vi "ReadPAQdata.vi"(4 "Tags":string[](array[string]), 6 "TableName":string, 8 "error in (no error)":errorcluster, 9 "Time-End":timestamp, 10 "Time-Start":timestamp, 11 "DBAL-BIN in":refnum<class "DBAL-BIN.lvclass">) -> (0 "error out":errorcluster, 2 "PAQ_section":T1, 3 "DBAL-BIN out":refnum<class "DBAL-BIN.lvclass">)   [LabVIEW 2020, in "Sgraph_lib_V1.lvlib" / "DBAL-BIN.lvclass"]
doc: "Andre Koelewijn, 8 May 2021,\n\nRead a PAQ TAGs from the BIN database for a defined time span.\nThe Layer input defines from which layer the data should be read."
uses:
  DBAL-BIN.lvclass
  controls/BIN/BINdata.ctl
  DBAL-BIN.lvclass/DBAL-BIN.ctl
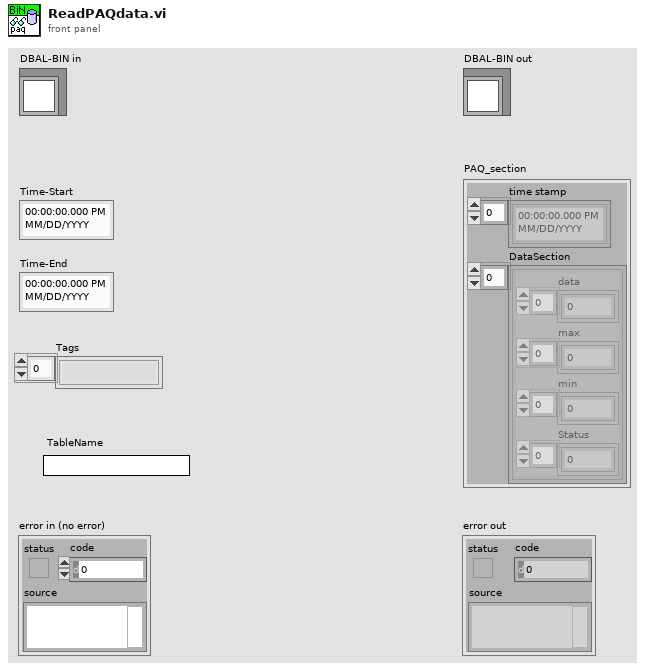
[diagram p1: front panel]
types:
  T1 = cluster{"time stamp":timestamp[], "DataSection":cluster{"data":dbl[], "max":dbl[], "min":dbl[], "Status":u32[]}[]}
  T2 = typedef "Sgraph_lib_V1.lvlib/DBAL-BIN.lvclass/BINdata.ctl" = cluster{"time":dbl[], "TagsData":cluster{"data":dbl[], "max":dbl[], "min":dbl[], "status":u32[]}[]}
  T3 = typedef "Sgraph_lib_V1.lvlib/DBAL-BIN.lvclass/BinFolderPace.ctl" = enum16{"PerDay", "PerWeek", "PerYear"}
  T4 = cluster{"Seq":i32, "Start":timestamp, "Stop":timestamp}[]
  T5 = cluster{"data":dbl[], "max":dbl[], "min":dbl[], "status":u32[]}[]
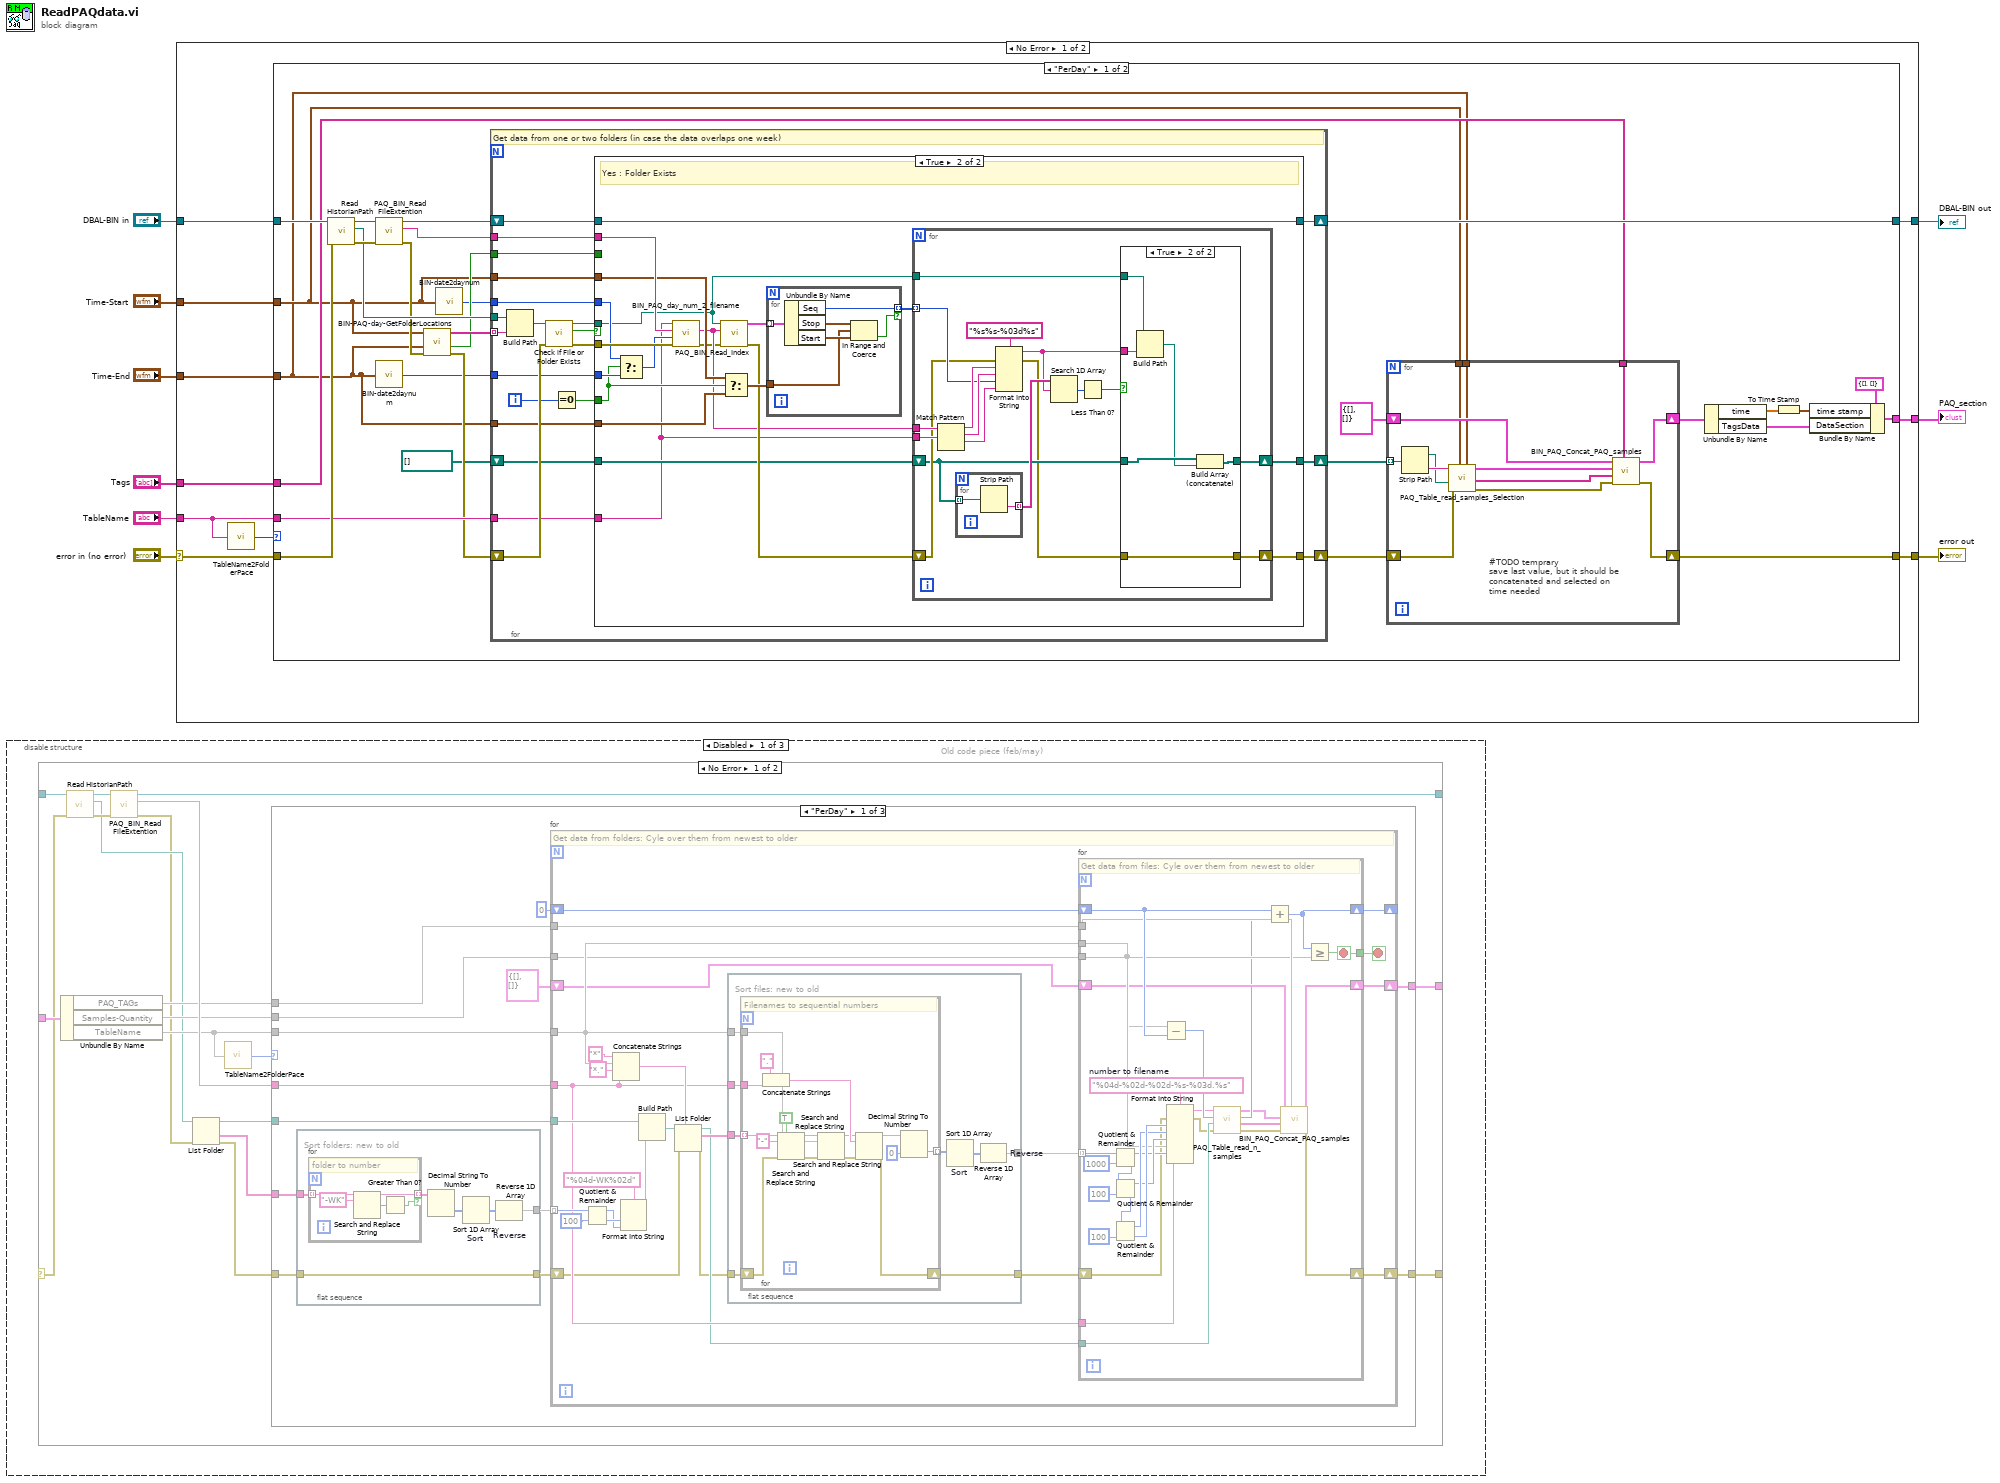
[diagram p0: block diagram]
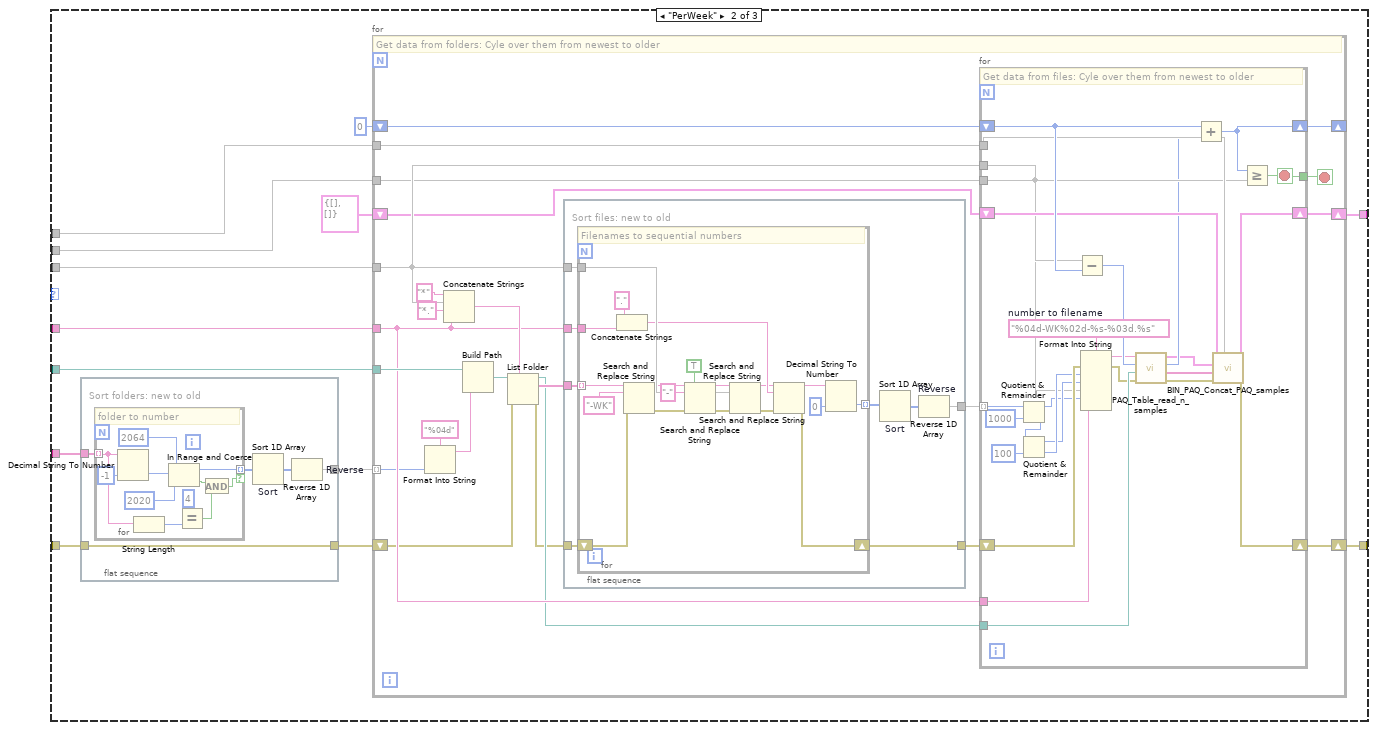
[diagram p2: hidden frame]
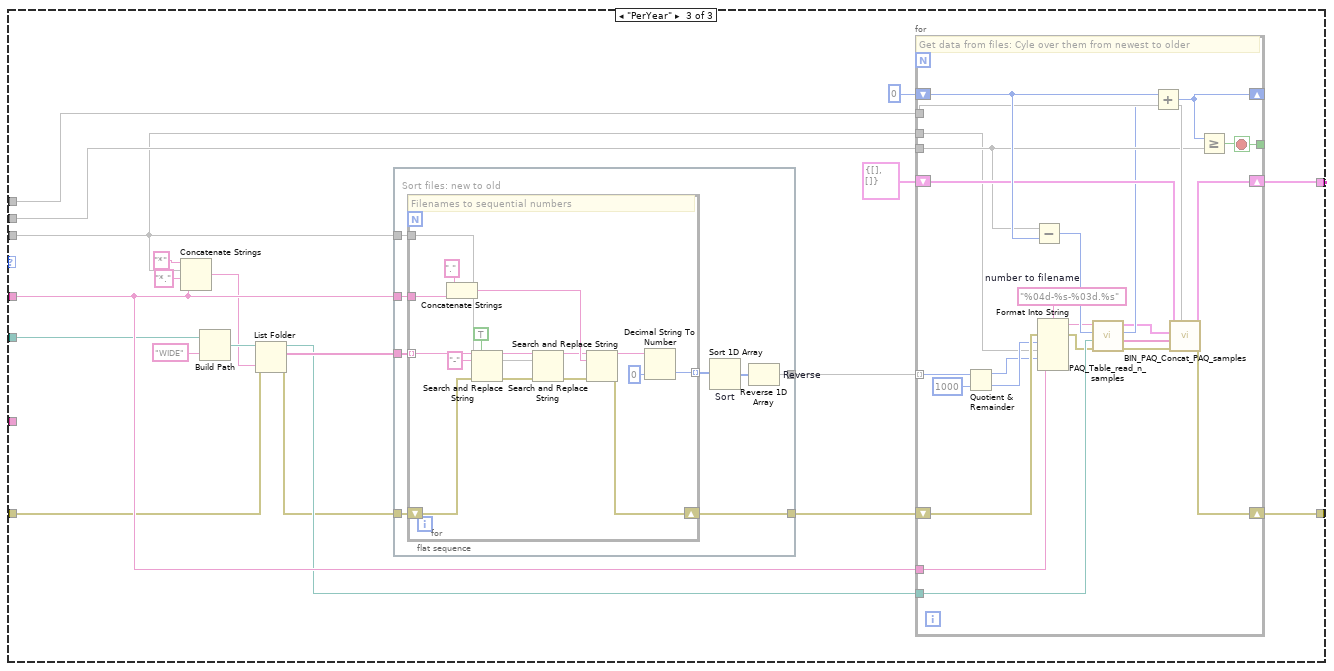
[diagram p3: hidden frame]
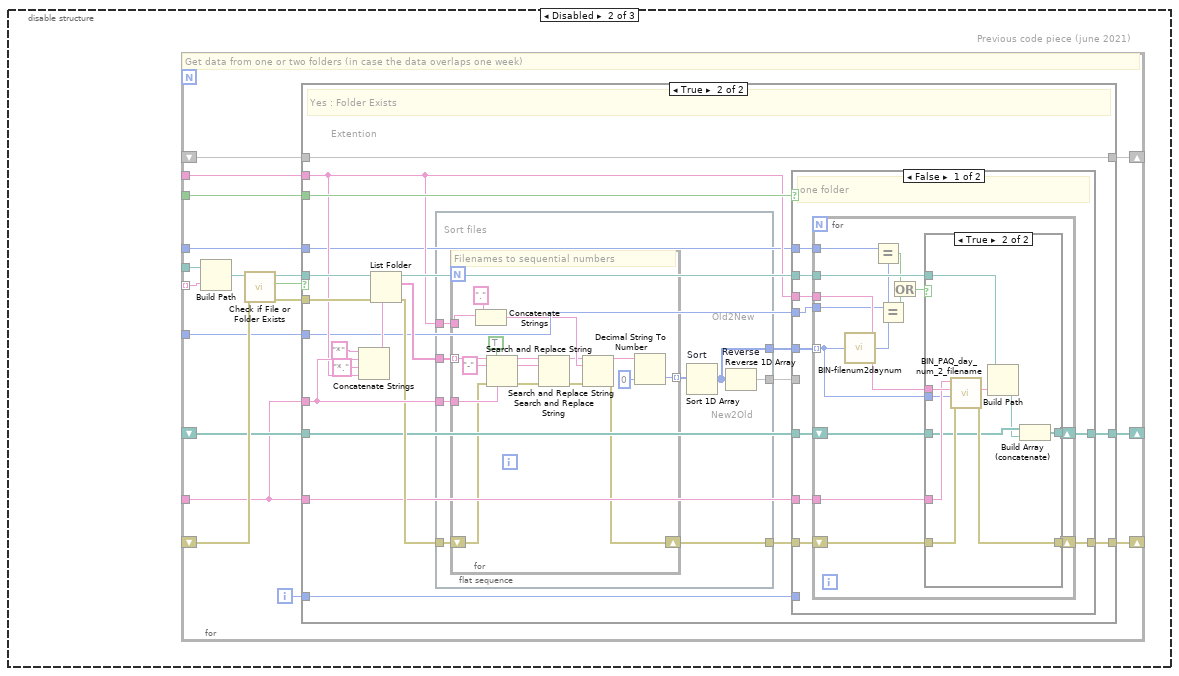
[diagram p5: hidden frame]
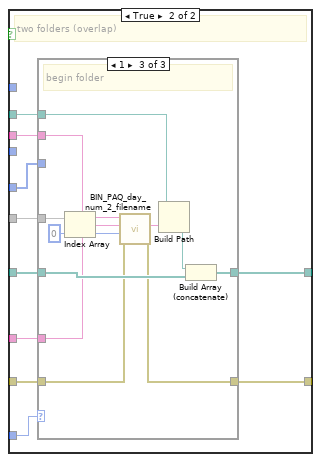
[diagram p8: hidden frame]
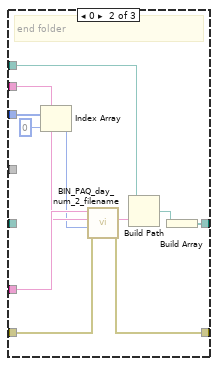
[diagram p10: hidden frame]
diagram:
  n1 = disable-structure shown="Disabled" {
    frame Disabled {
      # "Old code piece (feb/may)"
      n2 = case shown="No Error" {
        selector: _ -> [w22 w308]
        tunnel: [w26 w308] -> _
        tunnel: _ -> [w23 w309]
        tunnel: [w19 w309] -> _
        tunnel: _ -> [w27 _]
        tunnel: [w17 _] -> _
        frame No Error {
          n3 = Unbundle By Name(w27) -> ("PAQ_TAGs"=w18, "Samples-Quantity"=w20, "TableName"=w16)
          n4 = call "Read HistorianPath.vi"("error in (no error)"=w22, "DBAL-BIN in"=w23) -> ("error out"=w21:errorcluster, "HistorianPath"=w14:path, "DBAL-BIN out"=w24:refnum<class "DBAL-BIN.lvclass">)  [unwired: 7 in]
          n5 = call "PAQ_BIN_Read FileExtention.vi"("error in (no error)"=w21, "DBAL-BIN in"=w24) -> ("error out"=w13:errorcluster, "FileExtention"=w25:string, "DBAL-BIN out"=w19:refnum<class "DBAL-BIN.lvclass">)  [unwired: 7 in]
          n6 = List Folder(path=w14, error in=w13) -> (path out=w10:path, folder names=w12:string[], error out=w11:errorcluster)  [unwired: 2 in, 1 out]
          n7 = call "TableName2FolderPace.vi"("TableName"=w16) -> ("FolderPace"=w15:T3)  [unwired: 6 in]
          n8 = case shown="\"PerDay\"" w15 {
            tunnel: [w40 w145 w259] -> w26
            tunnel: w25 -> [w39 w144 w258]
            tunnel: w20 -> [w38 w143 w257]
            tunnel: w18 -> [w36 w141 w256]
            tunnel: [w34 w139 w254] -> w17
            tunnel: w16 -> [w33 w138 w253]
            tunnel: w12 -> [w32 w137 _]
            tunnel: w11 -> [w30 w135 w240]
            tunnel: w10 -> [w29 w134 w252]
            frame "PerDay" {
              n9 = flat-sequence {
                tunnel: w32 -> [w46]
                tunnel: [w41] -> w28
                tunnel: w30 -> [w43]
                tunnel: [w43] -> w31
                frame #0 {
                  # "Sort folders: new to old"
                  n10 = for {
                    tunnel: w46 -> [w51] mode=indexing
                    tunnel: [w49] -> w45 mode=indexing if=w47
                    # "folder to number"
                    n11 = Search and Replace String(input string=w51, search string="-WK") -> (result string=w49:string, number of replacements=w48:i32)  [unwired: 6 in, 2 out]
                    n12 = Greater Than 0?(x=w48) -> (x > 0?=w47:bool)
                  }
                  n13 = Decimal String To Number ("to num")(string=w45) -> (number=w44:i32[])  [unwired: 2 in, 1 out]
                  n14 = Sort 1D Array "Sort"(array=w44) -> (sorted array=w42:i32[])
                  n15 = Reverse 1D Array "Reverse"(array=w42) -> (reversed array=w41:i32[])
                }
              }
              n16 = for {
                shift-right: [w62] -> w40
                shift-left: w31 -> [w53]
                tunnel: w28 -> [w78] mode=indexing
                tunnel: w39 -> [w65]
                tunnel: w29 -> [w73]
                tunnel: w33 -> [w66]
                tunnel: w38 -> [w61]
                shift-right: [w59] -> _
                shift-left: 0 ("Fetched samples") -> [w60]
                tunnel: w36 -> [w58]
                shift-right: [w57] -> w34
                shift-left: T2 {"time"=[], "TagsData"=[]} ("BinHistData") -> [w56]
                stop <- w55 stop-if-true
                # "Get data from folders: Cyle over them from newest to older"
                n17 = Quotient & Remainder(x=w78, y=100) -> (x-y*floor(x/y)=w74:i32, floor(x/y)=w75:i32)
                n18 = Concatenate Strings("*", w66, "*.", w65) -> (w69:string)
                n19 = Format Into String(format string="%04d-WK%02d", w75, w74) -> (resulting string=w54:string)  [unwired: 2 in, 1 out]
                n20 = Build Path(base path=w73, name or relative path=w54) -> (appended path=w72:path)
                n21 = List Folder(path=w72, pattern=w69, error in=w53) -> (path out=w64:path, filenames=w67:string[], error out=w52:errorcluster)  [unwired: 1 in, 1 out]
                n22 = flat-sequence {
                  tunnel: w67 -> [w116]
                  tunnel: w66 -> [w115]
                  tunnel: w65 -> [w114]
                  tunnel: [w111] -> w68
                  tunnel: w52 -> [w110]
                  tunnel: [w109] -> w63
                  frame #0 {
                    # "Sort files: new to old"
                    n23 = for {
                      tunnel: w116 -> [w121] mode=indexing
                      tunnel: w115 -> [w129]
                      tunnel: w114 -> [w128]
                      tunnel: [w123] -> w112 mode=indexing
                      shift-right: [w117] -> w109
                      shift-left: w110 -> [w120]
                      # "Filenames to sequential numbers"
                      n24 = Concatenate Strings("." ("string"), w128) -> (w127:string)
                      n25 = Search and Replace String(replace all?=TRUE ("replace all? (F)"), input string=w121, search string="-", error in=w120) -> (result string=w130:string, error out=w119:errorcluster)  [unwired: 4 in, 2 out]
                      n26 = Search and Replace String(input string=w130, search string=w129, error in=w119) -> (result string=w126:string, error out=w118:errorcluster)  [unwired: 5 in, 2 out]
                      n27 = Search and Replace String(input string=w126, search string=w127, error in=w118) -> (result string=w124:string, error out=w117:errorcluster)  [unwired: 5 in, 2 out]
                      n28 = Decimal String To Number(string=w124, default (0L)=u64 0 ("default (0 I32)")) -> (number=w123:u64)  [unwired: 1 in, 1 out]
                    }
                    n29 = Sort 1D Array "Sort"(array=w112) -> (sorted array=w113:u64[])
                    n30 = Reverse 1D Array "Reverse"(array=w113) -> (reversed array=w111:u64[])
                  }
                }
                n31 = for {
                  tunnel: w68 -> [w107] mode=indexing
                  tunnel: w66 -> [w98]
                  tunnel: w65 -> [w96]
                  tunnel: w64 -> [w94]
                  shift-right: [w87] -> w62
                  shift-left: w63 -> [w95]
                  tunnel: w61 -> [w84]
                  shift-right: [w80] -> w59
                  shift-left: w60 -> [w91]
                  tunnel: w58 -> [w85]
                  shift-right: [w89] -> w57
                  shift-left: w56 -> [w90]
                  tunnel: [w83] -> w55
                  stop <- w83 stop-if-true
                  w102 = "%04d-%02d-%02d-%s-%03d.%s"  # number to filename
                  # "Get data from files: Cyle over them from newest to older"
                  n32 = Quotient & Remainder(x=w107, y=u64 1000) -> (x-y*floor(x/y)=w97:u64, floor(x/y)=w105:u64)
                  n33 = Quotient & Remainder(x=w105, y=u64 100) -> (x-y*floor(x/y)=w99:u64, floor(x/y)=w103:u64)
                  n34 = Quotient & Remainder(x=w103, y=u64 100) -> (x-y*floor(x/y)=w100:u64, floor(x/y)=w101:u64)
                  n35 = Subtract(x=w84, y=w91) -> (x-y=w92:i32)
                  n36 = Format Into String(format string=w102, error in=w95, w101, w100, w99, w98, w97, w96) -> (resulting string=w79:string, error out=w93:errorcluster)  [unwired: 1 in]
                  n37 = call "PAQ_Table_read_n_samples.vi"("error in (no error)"=w93, "Sub Path"=w94, "Required samples"=w92, "Table Filename"=w79) -> ("error out"=w88:errorcluster, "TAGs"=w86:string[], "Fetched samples"=w82:i32, "value"=w81:T2)  [unwired: 4 in]
                  n38 = Add(x=w91, y=w82) -> (x+y=w80:i32)
                  n39 = call "BIN_PAQ_Concat_PAQ_samples.vi"("Memory TAGs"=w85, "error in (no error)"=w88, "Added samples TAGs"=w86, "PAQ Samples to ADD"=w81, "PAQ Samples IN"=w90) -> ("error out"=w87:errorcluster, "PAQ Samples OUT"=w89:T2)  [unwired: 5 in]
                  n40 = Greater Or Equal?(x=w80, y=w84) -> (x >= y?=w83:bool)
                }
              }
            }
            frame "PerWeek" {
              n41 = flat-sequence {
                tunnel: w137 -> [w150]
                tunnel: [w147] -> w133
                tunnel: w135 -> [w149]
                tunnel: [w149] -> w136
                frame #0 {
                  # "Sort folders: new to old"
                  n42 = for {
                    tunnel: w150 -> [w156] mode=indexing
                    tunnel: [w157] -> w146 mode=indexing if=w151
                    # "folder to number"
                    n43 = Decimal String To Number ("to num")(string=w156, default (0L)=-1 ("default (0 I32)")) -> (number=w160:i32)  [unwired: 1 in, 1 out]
                    n44 = String Length(string=w156) -> (length=w155:i32)
                    n45 = In Range and Coerce(upper limit=2064 ("lower limit"), x=w160, lower limit=2020) -> (coerced(x)=w157:i32, In Range?=w153:bool)
                    n46 = Equal?(x=4, y=w155) -> (x = y?=w152:bool)
                    n47 = And(x=w153, y=w152) -> (x .and. y?=w151:bool)
                  }
                  n48 = Sort 1D Array "Sort"(array=w146) -> (sorted array=w148:i32[])
                  n49 = Reverse 1D Array "Reverse"(array=w148) -> (reversed array=w147:i32[])
                }
              }
              n50 = for {
                shift-right: [w173] -> w145
                shift-left: w136 -> [w163]
                tunnel: w133 -> [w164] mode=indexing
                tunnel: w144 -> [w176]
                tunnel: w134 -> [w184]
                tunnel: w138 -> [w177]
                tunnel: w143 -> [w172]
                shift-right: [w170] -> _
                shift-left: 0 ("Fetched samples") -> [w171]
                tunnel: w141 -> [w169]
                shift-right: [w168] -> w139
                shift-left: T2 {"time"=[], "TagsData"=[]} ("BinHistData") -> [w167]
                stop <- w166 stop-if-true
                # "Get data from folders: Cyle over them from newest to older"
                n51 = Format Into String(format string="%04d", w164) -> (resulting string=w165:string)  [unwired: 2 in, 1 out]
                n52 = Concatenate Strings("*", w177, "*.", w176) -> (w180:string)
                n53 = Build Path(base path=w184, name or relative path=w165) -> (appended path=w183:path)
                n54 = List Folder(path=w183, pattern=w180, error in=w163) -> (path out=w175:path, filenames=w178:string[], error out=w162:errorcluster)  [unwired: 1 in, 1 out]
                n55 = flat-sequence {
                  tunnel: w178 -> [w220]
                  tunnel: w177 -> [w219]
                  tunnel: w176 -> [w218]
                  tunnel: [w215] -> w179
                  tunnel: w162 -> [w214]
                  tunnel: [w213] -> w174
                  frame #0 {
                    # "Sort files: new to old"
                    n56 = for {
                      tunnel: w220 -> [w229] mode=indexing
                      tunnel: w219 -> [w237]
                      tunnel: w218 -> [w236]
                      tunnel: [w231] -> w216 mode=indexing
                      shift-right: [w221] -> w213
                      shift-left: w214 -> [w225]
                      # "Filenames to sequential numbers"
                      n57 = Concatenate Strings("." ("string"), w236) -> (w235:string)
                      n58 = Search and Replace String(input string=w229, search string="-WK", error in=w225) -> (result string=w227:string, error out=w224:errorcluster)  [unwired: 5 in, 2 out]
                      n59 = Search and Replace String(replace all?=TRUE ("replace all? (F)"), input string=w227, search string="-", error in=w224) -> (result string=w238:string, error out=w223:errorcluster)  [unwired: 4 in, 2 out]
                      n60 = Search and Replace String(input string=w238, search string=w237, error in=w223) -> (result string=w234:string, error out=w222:errorcluster)  [unwired: 5 in, 2 out]
                      n61 = Search and Replace String(input string=w234, search string=w235, error in=w222) -> (result string=w232:string, error out=w221:errorcluster)  [unwired: 5 in, 2 out]
                      n62 = Decimal String To Number(string=w232, default (0L)=u64 0 ("default (0 I32)")) -> (number=w231:u64)  [unwired: 1 in, 1 out]
                    }
                    n63 = Sort 1D Array "Sort"(array=w216) -> (sorted array=w217:u64[])
                    n64 = Reverse 1D Array "Reverse"(array=w217) -> (reversed array=w215:u64[])
                  }
                }
                n65 = for {
                  tunnel: w179 -> [w211] mode=indexing
                  tunnel: w177 -> [w189]
                  tunnel: w176 -> [w187]
                  tunnel: w175 -> [w206]
                  shift-right: [w199] -> w173
                  shift-left: w174 -> [w207]
                  tunnel: w172 -> [w196]
                  shift-right: [w192] -> w170
                  shift-left: w171 -> [w203]
                  tunnel: w169 -> [w197]
                  shift-right: [w201] -> w168
                  shift-left: w167 -> [w202]
                  tunnel: [w195] -> w166
                  stop <- w195 stop-if-true
                  w208 = "%04d-WK%02d-%s-%03d.%s"  # number to filename
                  # "Get data from files: Cyle over them from newest to older"
                  n66 = Quotient & Remainder(x=w211, y=u64 1000) -> (x-y*floor(x/y)=w188:u64, floor(x/y)=w209:u64)
                  n67 = Quotient & Remainder(x=w209, y=u64 100) -> (x-y*floor(x/y)=w190:u64, floor(x/y)=w191:u64)
                  n68 = Subtract(x=w196, y=w203) -> (x-y=w204:i32)
                  n69 = Format Into String(format string=w208, error in=w207, w191, w190, w189, w188, w187) -> (resulting string=w186:string, error out=w205:errorcluster)  [unwired: 1 in]
                  n70 = call "PAQ_Table_read_n_samples.vi"("error in (no error)"=w205, "Sub Path"=w206, "Required samples"=w204, "Table Filename"=w186) -> ("error out"=w200:errorcluster, "TAGs"=w198:string[], "Fetched samples"=w194:i32, "value"=w193:T2)  [unwired: 4 in]
                  n71 = Add(x=w203, y=w194) -> (x+y=w192:i32)
                  n72 = call "BIN_PAQ_Concat_PAQ_samples.vi"("Memory TAGs"=w197, "error in (no error)"=w200, "Added samples TAGs"=w198, "PAQ Samples to ADD"=w193, "PAQ Samples IN"=w202) -> ("error out"=w199:errorcluster, "PAQ Samples OUT"=w201:T2)  [unwired: 5 in]
                  n73 = Greater Or Equal?(x=w192, y=w196) -> (x >= y?=w195:bool)
                }
              }
            }
            frame "PerYear" {
              n74 = Concatenate Strings("*", w253, "*.", w258) -> (w248:string)
              n75 = Build Path(base path=w252, name or relative path="WIDE" ("format string")) -> (appended path=w251:path)
              n76 = List Folder(path=w251, pattern=w248, error in=w240) -> (path out=w245:path, filenames=w246:string[], error out=w241:errorcluster)  [unwired: 1 in, 1 out]
              n77 = flat-sequence {
                tunnel: w246 -> [w291]
                tunnel: w253 -> [w290]
                tunnel: w258 -> [w289]
                tunnel: [w286] -> w247
                tunnel: w241 -> [w285]
                tunnel: [w284] -> w244
                frame #0 {
                  # "Sort files: new to old"
                  n78 = for {
                    tunnel: w291 -> [w292] mode=indexing
                    tunnel: w290 -> [w305]
                    tunnel: w289 -> [w304]
                    tunnel: [w299] -> w287 mode=indexing
                    shift-right: [w294] -> w284
                    shift-left: w285 -> [w293]
                    # "Filenames to sequential numbers"
                    n79 = Concatenate Strings("." ("string"), w304) -> (w303:string)
                    n80 = Search and Replace String(replace all?=TRUE ("replace all? (F)"), input string=w292, search string="-", error in=w293) -> (result string=w306:string, error out=w296:errorcluster)  [unwired: 4 in, 2 out]
                    n81 = Search and Replace String(input string=w306, search string=w305, error in=w296) -> (result string=w302:string, error out=w295:errorcluster)  [unwired: 5 in, 2 out]
                    n82 = Search and Replace String(input string=w302, search string=w303, error in=w295) -> (result string=w300:string, error out=w294:errorcluster)  [unwired: 5 in, 2 out]
                    n83 = Decimal String To Number(string=w300, default (0L)=u64 0 ("default (0 I32)")) -> (number=w299:u64)  [unwired: 1 in, 1 out]
                  }
                  n84 = Sort 1D Array "Sort"(array=w287) -> (sorted array=w288:u64[])
                  n85 = Reverse 1D Array "Reverse"(array=w288) -> (reversed array=w286:u64[])
                }
              }
              n86 = for {
                tunnel: w247 -> [w282] mode=indexing
                tunnel: w253 -> [w262]
                tunnel: w258 -> [w260]
                tunnel: w245 -> [w279]
                shift-right: [w272] -> w259
                shift-left: w244 -> [w280]
                tunnel: w257 -> [w269]
                shift-right: [w265] -> _
                shift-left: 0 ("Fetched samples") -> [w276]
                tunnel: w256 -> [w270]
                shift-right: [w274] -> w254
                shift-left: T2 {"time"=[], "TagsData"=[]} ("BinHistData") -> [w275]
                tunnel: [w268] -> _
                stop <- w268 stop-if-true
                w281 = "%04d-%s-%03d.%s"  # number to filename
                # "Get data from files: Cyle over them from newest to older"
                n87 = Quotient & Remainder(x=w282, y=u64 1000) -> (x-y*floor(x/y)=w261:u64, floor(x/y)=w263:u64)
                n88 = Subtract(x=w269, y=w276) -> (x-y=w277:i32)
                n89 = Format Into String(format string=w281, error in=w280, w263, w262, w261, w260) -> (resulting string=w264:string, error out=w278:errorcluster)  [unwired: 1 in]
                n90 = call "PAQ_Table_read_n_samples.vi"("error in (no error)"=w278, "Sub Path"=w279, "Required samples"=w277, "Table Filename"=w264) -> ("error out"=w273:errorcluster, "TAGs"=w271:string[], "Fetched samples"=w267:i32, "value"=w266:T2)  [unwired: 4 in]
                n91 = Add(x=w276, y=w267) -> (x+y=w265:i32)
                n92 = call "BIN_PAQ_Concat_PAQ_samples.vi"("Memory TAGs"=w270, "error in (no error)"=w273, "Added samples TAGs"=w271, "PAQ Samples to ADD"=w266, "PAQ Samples IN"=w275) -> ("error out"=w272:errorcluster, "PAQ Samples OUT"=w274:T2)  [unwired: 5 in]
                n93 = Greater Or Equal?(x=w265, y=w269) -> (x >= y?=w268:bool)
              }
            }
          }
        }
        frame Error {
        }
      }
    }
    frame Disabled {
      # "Previous code piece (june 2021)"
      n94 = for {
        shift-right: [w320] -> _
        shift-left: _ -> [w324]
        shift-right: [w321] -> _
        shift-left: _ -> [w322]
        tunnel: _ -> [w326] mode=indexing
        tunnel: _ -> [w312]
        tunnel: _ -> [w327]
        tunnel: _ -> [w319]
        tunnel: _ -> [w316]
        shift-right: [w314] -> _
        shift-left: _ -> [w313]
        tunnel: _ -> [w310]
        tunnel: _ -> [w311]
        i -> [w315]
        # "Get data from one or two folders (in case the data overlaps one week)"
        n95 = Build Path(base path=w327, name or relative path=w326) -> (appended path=w325:path)
        n96 = call <vilib>:"Check if File or Folder Exists.vi"("error in (no error)"=w324, "path"=w325) -> ("error out"=w317:errorcluster, "file or folder exists?"=w323:bool, "dup path"=w318:path)  [unwired: 7 in]
        n97 = case shown="True" w323 {
          tunnel: w322 -> [w330 w352]
          tunnel: [w330 w352] -> w321
          tunnel: [w329 w336] -> w320
          tunnel: w312 -> [_ w345]
          tunnel: w319 -> [_ w334]
          tunnel: w318 -> [_ w348]
          tunnel: w317 -> [w329 w347]
          tunnel: w316 -> [_ w343]
          tunnel: w315 -> [_ w342]
          tunnel: [w328 w333] -> w314
          tunnel: w313 -> [w328 w339]
          tunnel: w312 -> [_ w335]
          tunnel: w311 -> [_ w332]
          tunnel: w310 -> [_ w331]
          frame False {
            # "No: Folder not found"
          }
          frame True {
            # "Extention"
            # "Yes : Folder Exists"
            n98 = Concatenate Strings("*", w345, "*.", w334) -> (w349:string)
            n99 = List Folder(path=w348, pattern=w349, error in=w347) -> (path out=w338:path, filenames=w346:string[], error out=w344:errorcluster)  [unwired: 1 in, 1 out]
            n100 = flat-sequence {
              tunnel: w346 -> [w431]
              tunnel: w345 -> [w430]
              tunnel: w334 -> [w429]
              tunnel: [w427] -> w340
              tunnel: w344 -> [w426]
              tunnel: [w425] -> w337
              tunnel: [w424] -> w341
              frame #0 {
                # "Old2New"
                # "New2Old"
                # "Sort files"
                n101 = for {
                  tunnel: w431 -> [w437] mode=indexing
                  tunnel: w430 -> [w445]
                  tunnel: w429 -> [w444]
                  tunnel: [w439] -> w428 mode=indexing
                  shift-right: [w433] -> w425
                  shift-left: w426 -> [w436]
                  # "Filenames to sequential numbers"
                  n102 = Concatenate Strings("." ("string"), w444) -> (w443:string)
                  n103 = Search and Replace String(replace all?=TRUE ("replace all? (F)"), input string=w437, search string="-", error in=w436) -> (result string=w432:string, error out=w435:errorcluster)  [unwired: 4 in, 2 out]
                  n104 = Search and Replace String(input string=w432, search string=w445, error in=w435) -> (result string=w442:string, error out=w434:errorcluster)  [unwired: 5 in, 2 out]
                  n105 = Search and Replace String(input string=w442, search string=w443, error in=w434) -> (result string=w440:string, error out=w433:errorcluster)  [unwired: 5 in, 2 out]
                  n106 = Decimal String To Number(string=w440, default (0L)=u64 0 ("default (0 I32)")) -> (number=w439:u64)  [unwired: 1 in, 1 out]
                }
                n107 = Sort 1D Array "Sort"(array=w428) -> (sorted array=w424:u64[])
                n108 = Reverse 1D Array "Reverse"(array=w424) -> (reversed array=w427:u64[])
              }
            }
            n109 = case shown="False" w343 {
              tunnel: w342 -> [_ w398]
              tunnel: w341 -> [w357 w397]
              tunnel: w340 -> [_ w396]
              tunnel: w339 -> [w360 w395]
              tunnel: w338 -> [w358 w394]
              tunnel: w337 -> [w362 w393]
              tunnel: [w361 w392] -> w336
              tunnel: w335 -> [w355 w391]
              tunnel: w334 -> [w356 w390]
              tunnel: [w359 w389] -> w333
              tunnel: w332 -> [w354 _]
              tunnel: w331 -> [w353 _]
              frame False {
                # "one folder"
                n110 = for {
                  shift-right: [w374] -> w361
                  shift-left: w362 -> [w375]
                  shift-right: [w370] -> w359
                  shift-left: w360 -> [w371]
                  tunnel: w358 -> [w376]
                  tunnel: w357 -> [w365] mode=indexing
                  tunnel: w356 -> [w373]
                  tunnel: w355 -> [w372]
                  tunnel: w354 -> [w369]
                  tunnel: w353 -> [w368]
                  n111 = call "BIN-filenum2daynum.vi"("FileNum"=w365) -> ("DayNum"=w364:u64)  [unwired: 8 in]
                  n112 = Equal?(x=w369, y=w364) -> (x = y?=w366:bool)
                  n113 = Equal?(x=w368, y=w364) -> (x = y?=w367:bool)
                  n114 = Or(x=w366, y=w367) -> (x .or. y?=w363:bool)
                  n115 = case shown="True" w363 {
                    tunnel: w376 -> [_ w388]
                    tunnel: w375 -> [w377 w387]
                    tunnel: [w377 w386] -> w374
                    tunnel: w373 -> [_ w384]
                    tunnel: w372 -> [_ w383]
                    tunnel: w371 -> [w378 w382]
                    tunnel: [w378 w380] -> w370
                    tunnel: w365 -> [_ w379]
                    frame False {
                    }
                    frame True {
                      n116 = call "BIN_PAQ_day_num_2_filename.vi"("error in"=w387, "num"=w379, "ext"=w384, "TableName"=w383) -> ("error out"=w386:errorcluster, "FileName"=w385:string)  [unwired: 6 in]
                      n117 = Build Path(base path=w388, name or relative path=w385) -> (appended path=w381:path)
                      n118 = Build Array (concatenate)(w382, w381) -> (w380:path[])
                    }
                  }
                }
              }
              frame True {
                # "two folders (overlap)"
                n119 = case shown="1" w398 {
                  tunnel: w397 -> [_ w411 _]
                  tunnel: [w400 w401 w422] -> w389
                  tunnel: w396 -> [_ _ w421]
                  tunnel: w395 -> [w400 _ w420]
                  tunnel: w394 -> [_ w409 w419]
                  tunnel: w393 -> [w399 w408 w417]
                  tunnel: [w399 w407 w416] -> w392
                  tunnel: w391 -> [_ w406 w415]
                  tunnel: w390 -> [_ w405 w414]
                  frame Default {
                    # "not used"
                  }
                  frame 0 {
                    # "end folder"
                    n120 = Index Array(array=w411, index=0) -> (element=w404:u64)
                    n121 = call "BIN_PAQ_day_num_2_filename.vi"("error in"=w408, "num"=w404, "ext"=w405, "TableName"=w406) -> ("error out"=w407:errorcluster, "FileName"=w403:string)  [unwired: 6 in]
                    n122 = Build Path(base path=w409, name or relative path=w403) -> (appended path=w402:path)
                    n123 = Build Array(w402) -> (w401:path[])
                  }
                  frame 1 {
                    # "begin folder"
                    n124 = Index Array(array=w421, index=0) -> (element=w418:u64)
                    n125 = call "BIN_PAQ_day_num_2_filename.vi"("error in"=w417, "num"=w418, "ext"=w414, "TableName"=w415) -> ("error out"=w416:errorcluster, "FileName"=w413:string)  [unwired: 6 in]
                    n126 = Build Path(base path=w419, name or relative path=w413) -> (appended path=w412:path)
                    n127 = Build Array (concatenate)(w412, w420) -> (w422:path[])
                  }
                }
              }
            }
          }
        }
      }
    }
    frame Enabled {
    }
  }
  n128 = case shown="No Error" "error in (no error)" {
    selector: "error in (no error)" -> [w454 w580]
    tunnel: [w453 w580] -> w8
    tunnel: [w455 w579] -> w6
    tunnel: "DBAL-BIN in" -> [w456 w579]
    tunnel: "Time-Start" -> [w451 _]
    tunnel: "Time-End" -> [w450 _]
    tunnel: "Tags" -> [w449 _]
    tunnel: "TableName" -> [w452 _]
    tunnel: [w448 _] -> w1
    frame No Error {
      n129 = call "TableName2FolderPace.vi"("TableName"=w452) -> ("FolderPace"=w457:T3)  [unwired: 6 in]
      n130 = case shown="\"PerDay\"" w457 {
        tunnel: w456 -> [w486 w578]
        tunnel: [w481 w578] -> w455
        tunnel: w454 -> [w483 w577]
        tunnel: [w468 w577] -> w453
        tunnel: w452 -> [w480 _]
        tunnel: w451 -> [w459 _]
        tunnel: w450 -> [w458 _]
        tunnel: w449 -> [w460 _]
        tunnel: [w461 _] -> w448
        frame "PerDay" {
          n131 = call "Read HistorianPath.vi"("error in (no error)"=w483, "DBAL-BIN in"=w486) -> ("error out"=w484:errorcluster, "HistorianPath"=w478:path, "DBAL-BIN out"=w485:refnum<class "DBAL-BIN.lvclass">)  [unwired: 7 in]
          n132 = call "PAQ_BIN_Read FileExtention.vi"("error in (no error)"=w484, "DBAL-BIN in"=w485) -> ("error out"=w477:errorcluster, "FileExtention"=w479:string, "DBAL-BIN out"=w482:refnum<class "DBAL-BIN.lvclass">)  [unwired: 7 in]
          n133 = call "BIN-date2daynum.vi"("Time"=w458) -> ("DayNum"=w471:u64)  [unwired: 8 in]
          n134 = call "BIN-PAQ-day-GetFolderLocations.vi"("error in (no error)"=w477, "Time-End"=w458, "Time-Start"=w459) -> ("error out"=w475:errorcluster, "Overlap?"=w474:bool, "Folders"=w476:string[])  [unwired: 6 in]
          n135 = call "BIN-date2daynum.vi"("Time"=w459) -> ("DayNum"=w470:u64)  [unwired: 8 in]
          n136 = for {
            shift-right: [w513] -> w469
            shift-left: w475 -> [w517]
            shift-right: [w514] -> w481
            shift-left: w482 -> [w515]
            tunnel: w476 -> [w519] mode=indexing
            tunnel: w480 -> [w506]
            tunnel: w478 -> [w520]
            tunnel: w479 -> [w512]
            tunnel: w474 -> [w509]
            shift-right: [w508] -> w472
            shift-left: path[] [] -> [w507]
            tunnel: w471 -> [w504]
            tunnel: w470 -> [w505]
            tunnel: w459 -> [w501]
            tunnel: w458 -> [w500]
            i -> [w503]
            # "Get data from one or two folders (in case the data overlaps one week)"
            n137 = Build Path(base path=w520, name or relative path=w519) -> (appended path=w518:path)
            n138 = call <vilib>:"Check if File or Folder Exists.vi"("error in (no error)"=w517, "path"=w518) -> ("error out"=w510:errorcluster, "file or folder exists?"=w516:bool, "dup path"=w511:path)  [unwired: 7 in]
            n139 = Equal To 0?(x=w503) -> (x = 0?=w502:bool)
            n140 = case shown="True" w516 {
              tunnel: w515 -> [w523 w541]
              tunnel: [w523 w541] -> w514
              tunnel: [w522 w531] -> w513
              tunnel: w512 -> [_ w543]
              tunnel: w511 -> [_ w525]
              tunnel: w510 -> [w522 w542]
              tunnel: w509 -> [_ _]
              tunnel: [w521 w528] -> w508
              tunnel: w507 -> [w521 w529]
              tunnel: w506 -> [_ w526]
              tunnel: w505 -> [_ w540]
              tunnel: w504 -> [_ w539]
              tunnel: w502 -> [_ w537]
              tunnel: w501 -> [_ w535]
              tunnel: w500 -> [_ w536]
              frame False {
                # "No: Folder not found"
              }
              frame True {
                # "Yes : Folder Exists"
                n141 = Select(t=w540, s=w537, f=w539) -> (s? t:f=w538:u64)
                n142 = call "BIN_PAQ_day_num_2_filename.vi"("error in"=w542, "num"=w538, "ext"=w543, "TableName"=w526) -> ("error out"=w524:errorcluster, "FileName"=w527:string)  [unwired: 6 in]
                n143 = call "PAQ_BIN_Read_Index.vi"("error in (no error)"=w524, "TableName"=w527, "Path"=w525) -> ("error out"=w532:errorcluster, "TimeStamps"=w534:T4)  [unwired: 7 in]
                n144 = Select(t=w535, s=w537, f=w536) -> (s? t:f=w533:timestamp)
                n145 = for {
                  tunnel: w534 -> [w576] mode=indexing
                  tunnel: w533 -> [w573]
                  tunnel: [w572] -> w530 mode=indexing if=w571
                  n146 = Unbundle By Name(w576) -> ("Seq"=w572:i32, "Stop"=w575:timestamp, "Start"=w574:timestamp)
                  n147 = In Range and Coerce(upper limit=w575, x=w573, lower limit=w574) -> (In Range?=w571:bool)  [unwired: 1 out]
                }
                n148 = for {
                  shift-right: [w544] -> w531
                  shift-left: w532 -> [w552]
                  tunnel: w530 -> [w555] mode=indexing
                  shift-right: [w546] -> w528
                  shift-left: w529 -> [w547]
                  tunnel: w527 -> [w560]
                  tunnel: w526 -> [w559]
                  tunnel: w525 -> [w548]
                  n149 = Match Pattern(string=w560, regular expression=w559) -> (before substring=w557:string, match substring=w556:string, after substring=w554:string)  [unwired: 1 in, 1 out]
                  n150 = for {
                    tunnel: w547 -> [w570] mode=indexing
                    tunnel: [w569] -> w553 mode=indexing
                    n151 = Strip Path(path=w570) -> (name=w569:string)  [unwired: 1 out]
                  }
                  n152 = Format Into String(format string="%s%s-%03d%s", error in=w552, w557, w556, w555, w554) -> (resulting string=w549:string, error out=w545:errorcluster)  [unwired: 1 in]
                  n153 = Search 1D Array(1D array=w553, element=w549) -> (index of element=w551:i32)  [unwired: 1 in]
                  n154 = Less Than 0?(x=w551) -> (x < 0?=w550:bool)
                  n155 = case shown="True" w550 {
                    tunnel: w549 -> [_ w567]
                    tunnel: w548 -> [_ w568]
                    tunnel: w547 -> [w562 w565]
                    tunnel: [w562 w563] -> w546
                    tunnel: w545 -> [w561 w566]
                    tunnel: [w561 w566] -> w544
                    frame False {
                    }
                    frame True {
                      n156 = Build Path(base path=w568, name or relative path=w567) -> (appended path=w564:path)
                      n157 = Build Array (concatenate)(w565, w564) -> (w563:path[])
                    }
                  }
                }
              }
            }
          }
          n158 = for {
            tunnel: w472 -> [w498] mode=indexing
            shift-right: [w489] -> w468
            shift-left: w469 -> [w499]
            shift-right: [w494] -> w462
            shift-left: T2 {"time"=[], "TagsData"=[]} ("BinHistData") -> [w495]
            tunnel: w460 -> [w492]
            tunnel: w459 -> [w488]
            tunnel: w458 -> [w487]
            # "#TODO temprary\nsave last value, but it should be\nconcatenated and selected on \ntime needed"
            n159 = Strip Path(path=w498) -> (stripped path=w496:path, name=w497:string)
            n160 = call "PAQ_Table_read_samples_Selection.vi"("Time-End"=w487, "Time-Start"=w488, "error in (no error)"=w499, "Sub Path"=w496, "Table Filename"=w497) -> ("error out"=w490:errorcluster, "TAGs"=w491:string[], "Fetched PAQ-samples"=w493:T2)  [unwired: 3 in, 1 out]
            n161 = call "BIN_PAQ_Concat_PAQ_samples.vi"("Memory TAGs"=w492, "error in (no error)"=w490, "Added samples TAGs"=w491, "PAQ Samples to ADD"=w493, "PAQ Samples IN"=w495) -> ("error out"=w489:errorcluster, "PAQ Samples OUT"=w494:T2)  [unwired: 5 in]
          }
          n162 = Unbundle By Name(w462) -> ("time"=w465:dbl[], "TagsData"=w466:T5)
          n163 = To Time Stamp(1:w465) -> (0:w464:timestamp[])
          n164 = Bundle By Name(cluster=T1 {"time stamp"=[], "DataSection"=[]} ("PAQ_section"), "time stamp"=w464, "DataSection"=w466) -> (w461:T1)
        }
        frame Default {
        }
      }
    }
    frame Error {
    }
  }
  "error out" <- w8
  "DBAL-BIN out" <- w6
  "PAQ_section" <- w1
